vi "Set_MultiVar_BulkMode_Values.vi"(8 "error in (no error)":errorcluster, 9 "varValues":dbl[][](array[numeric]) format="%#_13g", 10 "varNames":string[](array[string]), 11 "muExpr in":refnum<class "mupExpr.lvclass">) -> (0 "error out":errorcluster, 3 "muExpr out":refnum<class "mupExpr.lvclass">)   [LabVIEW 2015, in "mupExpr.lvclass"]
doc: "Set the bulk mode values for a list of variables.\n\nNote that the array of values provided for variable values should be of size:\nNum Rows: Number of Variables\nNum Cols: Bulk Size\n\nIf any variable is not found, a warning is generated."
uses:
  mupExpr.lvclass
  mupExpr.lvclass/mupExpr.ctl
  mupLib/mupSetVarValue_Array.vi
  <vilib>/Utility/error.llb/Error Cluster From Error Code.vi
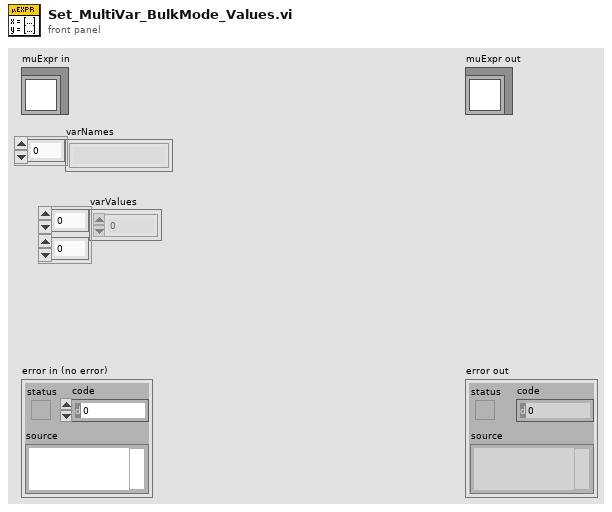
[diagram p1: front panel]
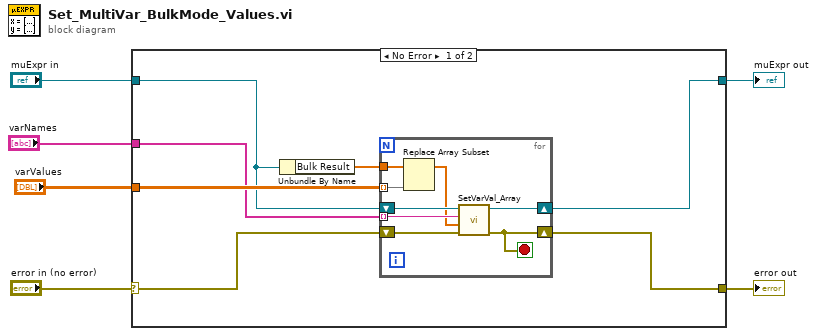
[diagram p0: block diagram]
diagram:
  n1 = case shown="No Error" "error in (no error)" {
    selector: "error in (no error)" -> [w7 w22]
    tunnel: "varValues" -> [w13 _]
    tunnel: "varNames" -> [w12 _]
    tunnel: "muExpr in" -> [w10 w23]
    tunnel: [w8 w22] -> w3
    tunnel: [w9 w23] -> w2
    frame No Error {
      n2 = Unbundle By Name(w10) -> ("Bulk Result"=w11:dbl[])
      n3 = for {
        tunnel: w12 -> [w21] mode=indexing
        tunnel: w11 -> [w18]
        tunnel: w13 -> [w17] mode=indexing
        shift-right: [w14] -> w8
        shift-left: w7 -> [w20]
        shift-right: [w15] -> w9
        shift-left: w10 -> [w19]
        stop <- w14 stop-if-true
        n4 = Replace Array Subset(array=w18, new element=w17) -> (w16:dbl[])  [unwired: 1 in]
        n5 = call "SetVarVal_Array.vi"("error in (no error)"=w20, "varValue"=w16, "varName"=w21, "muExpr in"=w19) -> ("error out"=w14:errorcluster, "muExpr out"=w15:refnum<class "mupExpr.lvclass">)  [unwired: 6 in]
      }
    }
    frame Error {
    }
  }
  "error out" <- w3
  "muExpr out" <- w2
